vi "SoundInput-DAQ.vi"(7 "Name(\"\" to use uuid)":string="Acquisition") -> ()   [LabVIEW 2017, in "SoundInput-DAQ.lvlib"]
uses:
  SoundInput-DAQ.lvlib
  <vilib>/sound2/lvsound2.llb/Sound Data Format.ctl
  <vilib>/sound2/lvsound2.llb/Sampling Mode.ctl
  bc6f9ce3-7135-4df3-9fce-67397201bd09.vi
  15320dbe-bea9-49cb-a904-6d9e4fcf93d5.vi
  f3e3012a-dc83-45d7-82c5-490bef76f43f.vi
  e2413101-be31-4c43-921b-7e7496268bc5.vi
  07cbb487-6694-43fd-ac53-f2be3466fcff.vi
  fecb174d-6823-407c-a974-ffebb4610b14.vi
  0bf643a1-791c-4b4c-b91f-da80b9c7e2fb.vi
  041ba748-83ae-40d3-86c4-8e2f4b565384.vi
  <userlib>/_NEVSTOP/Communicable State Machine(CSM)/AdvanceAPI/CSM - Revert Arguments-Safe String.vi
  <userlib>/_NEVSTOP/Communicable State Machine(CSM)/_Shared/Trim Single-line Text.vi
  <userlib>/_NEVSTOP/Communicable State Machine(CSM)/AdvanceAPI/CSM - Make String Arguments Safe.vi
  <userlib>/_NEVSTOP/Communicable State Machine(CSM)/AdvanceAPI/CSM - Break Down Multiple States String.vi
  <userlib>/_NEVSTOP/Communicable State Machine(CSM)/AdvanceAPI/CSM - Compact Multiple States.vi
  f3e3012a-dc83-45d7-82c5-490bef76f43f.vi/99de0c97-112a-4c86-9094-c187659127e1.vi
  <userlib>/_NEVSTOP/Communicable State Machine(CSM)/Utility/Build Error Cluster.vi
  0bf643a1-791c-4b4c-b91f-da80b9c7e2fb.vi/99de0c97-112a-4c86-9094-c187659127e1.vi
  <userlib>/_NEVSTOP/Communicable State Machine(CSM)/AdvanceAPI/CSM - Keywords.vi
  <vilib>/Utility/Data Type/Get Type Information.vi
  <userlib>/_NEVSTOP/Communicable State Machine(CSM)/addons/API-String-Arugments-Support/_Support/Data To SingleElementsArray_csm.vi
  <userlib>/_NEVSTOP/Communicable State Machine(CSM)/addons/API-String-Arugments-Support/_Support/Data To API String Arguments.vi
  <userlib>/_NEVSTOP/Communicable State Machine(CSM)/addons/INI-Static-Variable-Support/_Support/Parse Used Session and Name.vi
  <userlib>/_NEVSTOP/Communicable State Machine(CSM)/addons/INI-Static-Variable-Support/_Support/INI-FGV(lvlibp).vi
  <userlib>/_NEVSTOP/Communicable State Machine(CSM)/addons/INI-Static-Variable-Support/_Support/Populate String with INI Variable.vi
  <userlib>/_NEVSTOP/Communicable State Machine(CSM)/addons/API-String-Arugments-Support/_Support/Convert API String Arguments to Data(variant).vi
  <userlib>/_NEVSTOP/Communicable State Machine(CSM)/addons/API-String-Arugments-Support/_Support/SingleElementsArray To Data_csm.vi
  <userlib>/_NEVSTOP/Communicable State Machine(CSM)/addons/API-String-Arugments-Support/_Support/Query Data as API String Arguments(variant).vi
  <vilib>/sound2/lvsound2.llb/Sound Input Read (DBL).vi
  <userlib>/_NEVSTOP/Communicable State Machine(CSM)/addons/MassData-Parameter/_support/FGV-MassData(lvlibp).vi
  <userlib>/_NEVSTOP/Communicable State Machine(CSM)/_Polymophic/Add State(s) to Queue By BOOL(Element).vi
  <userlib>/_NEVSTOP/Communicable State Machine(CSM)/_Polymophic/CSM - Filter Duplicated Lines.vi
  <userlib>/_NEVSTOP/Communicable State Machine(CSM)/_Polymophic/CSM - Replace Marks in Messages.vi
  <userlib>/_NEVSTOP/Communicable State Machine(CSM)/Communicable State Machine.lvlib
  <userlib>/_NEVSTOP/Communicable State Machine(CSM)/addons/Loop-Support/CSM Loop Support.lvlib
  <userlib>/_NEVSTOP/Communicable State Machine(CSM)/_Shared/CSM Shared.lvlib
panel:
  in  "Sound Format":T1={"sample rate (S/s)"=20000.0, "number of channels"=2, "bits per sample"=16}
  in  "Device ID":u32 format="%.0x"
  in  "SamplePeroid(ms)":i32=200
  out "Raw Data":waveform(dbl)[](graph)
  in  "Cancel Button":bool
  in  "OK Button":bool
  out "Error Occurred":errorcluster
  out "State History":string
  # "*(Windows) You must have DirectX 8.0 or later to use the Sound VIs. (Linux) You must have the Open Sound System (OSS) driver to use the Sound VIs."
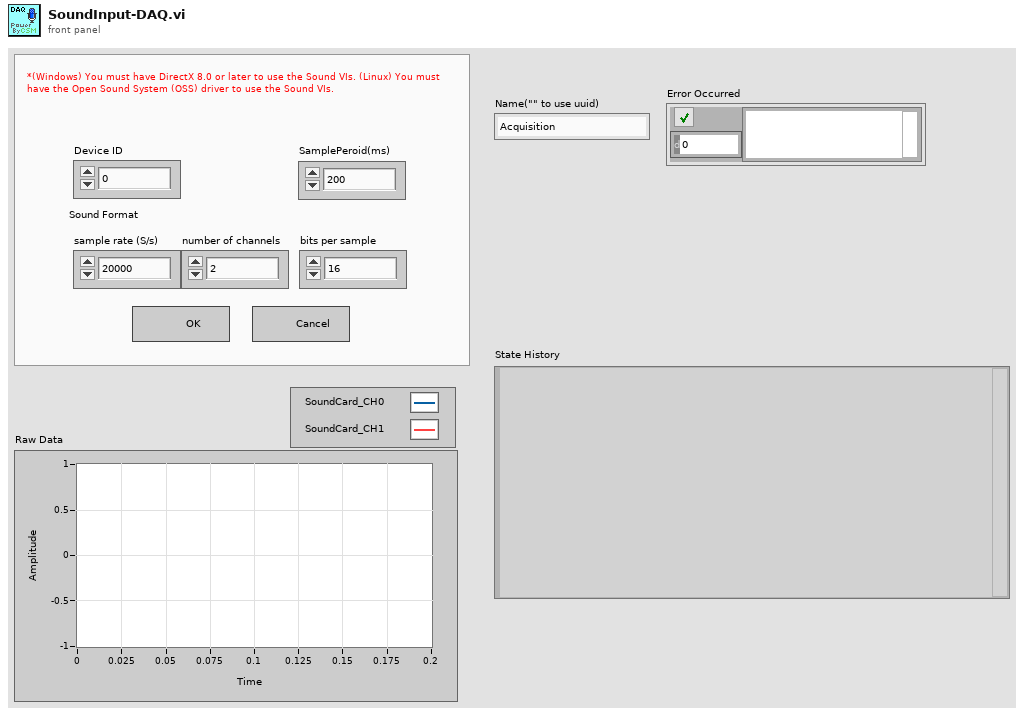
[diagram p1: front panel]
types:
  T1 = cluster{"sample rate (S/s)":dbl, "number of channels":i32, "bits per sample":i32}
  T2 = enum32{"Invalid", "Default", "Floating", "Floating/Auto-Hide", "Modal"}
  T3 = cluster{"Device ID":u32, "SamplePeroid(ms)":i32, "Sound Format":cluster{"sample rate (S/s)":dbl, "number of channels":i32, "bits per sample":i32}}
  T4 = enum32{"Invalid", "Standard", "Closed", "Hidden", "Minimized", "Maximized"}
  T5 = enum32{"invalid app kind", "Development System", "Run Time System", "Student Edition", "Embedded LabVIEW", "Evaluation", "Custom"}
  T6 = typedef "Communicable State Machine.lvlib/_CSM_Response Source Message.ctl" = cluster{"‘State":string, "’Arguments":string, "’Error":errorcluster}
  T7 = cluster{"Current VI Reference":refnum<vi>, "Close Panel on Exit?":bool}
  T8 = typedef "Sound Data Format.ctl" = cluster{"sample rate (S/s)":dbl, "number of channels":i32, "bits per sample":i32}
  T9 = cluster{"Core":cluster{"Current VI Reference":refnum<vi>, "Close Panel on Exit?":bool}, "Configuration":cluster{"Device ID":u32, "SamplePeroid(ms)":i32, "Sound Format":T8}, "State":enum16{"Idle", "Acquiring"}, "Number of Samples/ch":i32, "timestamp":timestamp}
  T10 = cluster{"Device ID":u32, "SamplePeroid(ms)":i32, "Sound Format":T8}
  T11 = typedef "Sampling Mode.ctl" = i32
  T12 = typedef "Sound Input Task ID.ctl" = u32
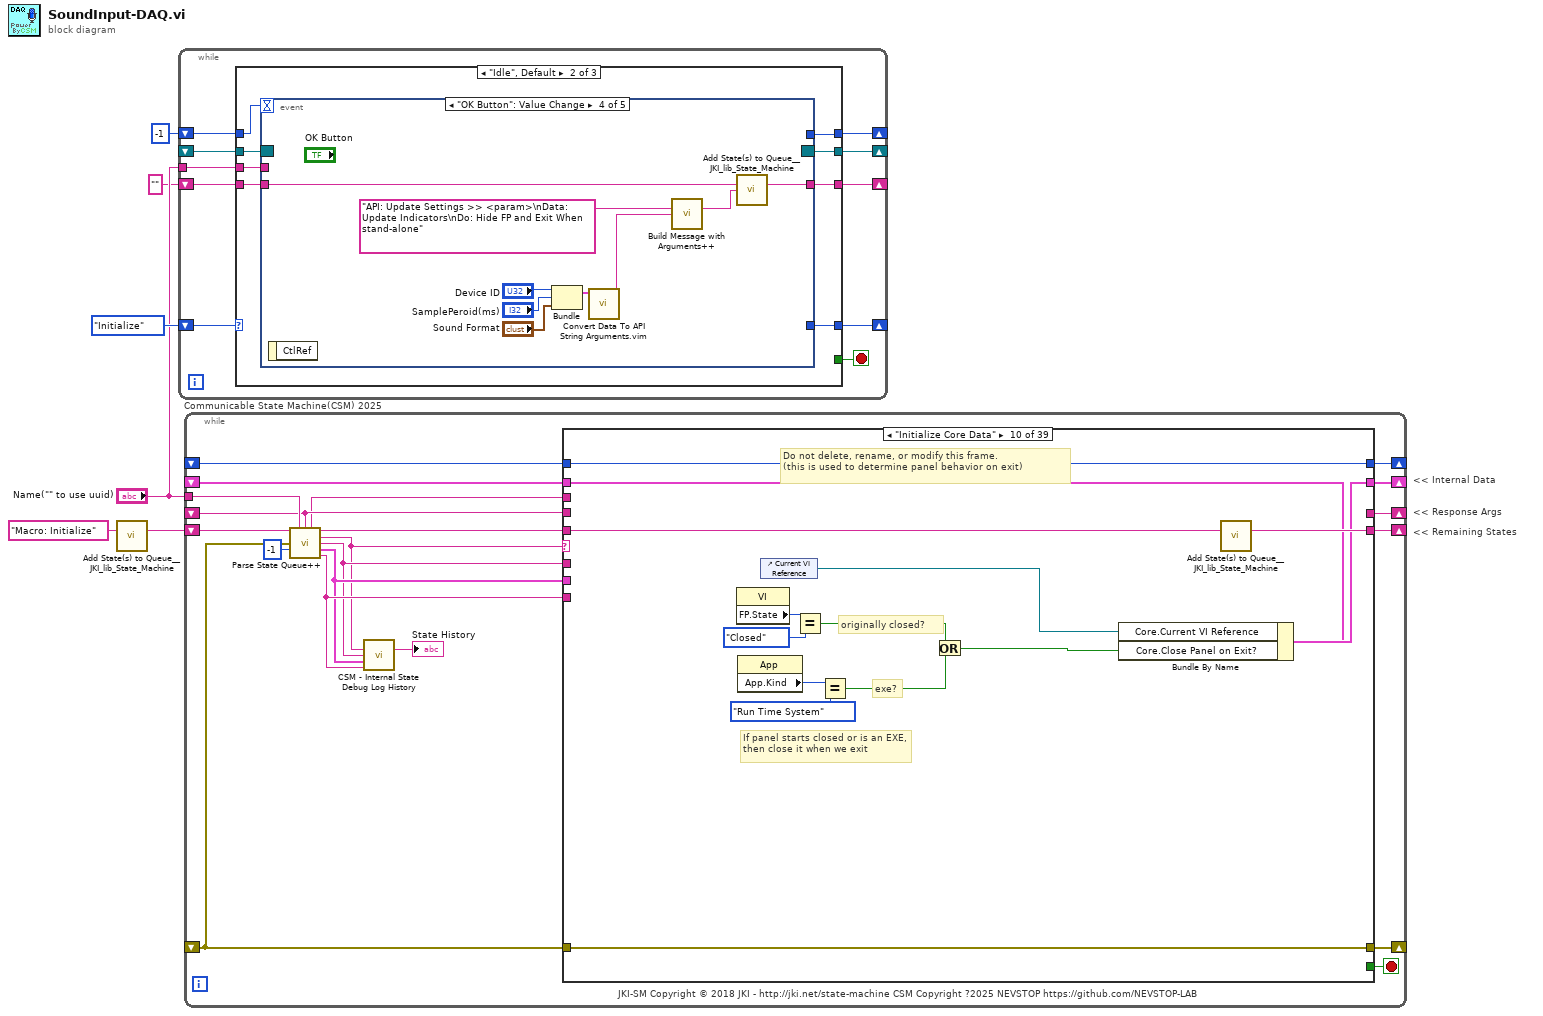
[diagram p0: block diagram]
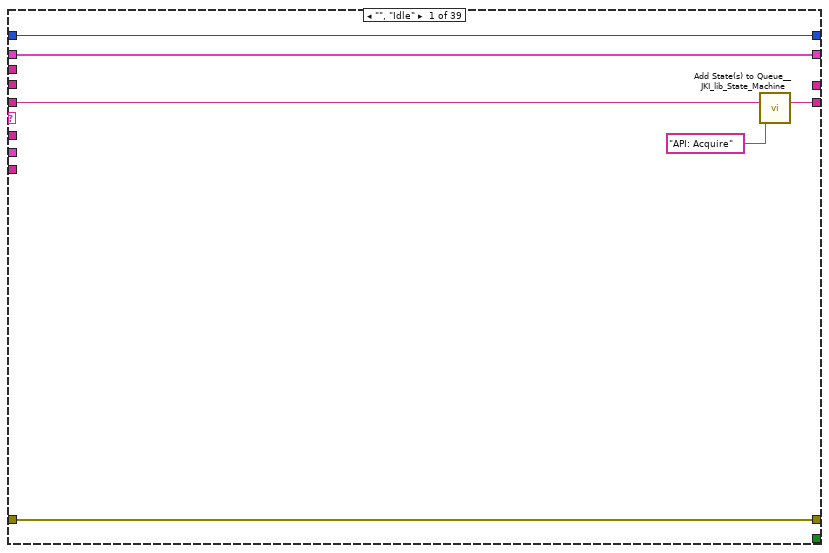
[diagram p2: hidden frame]
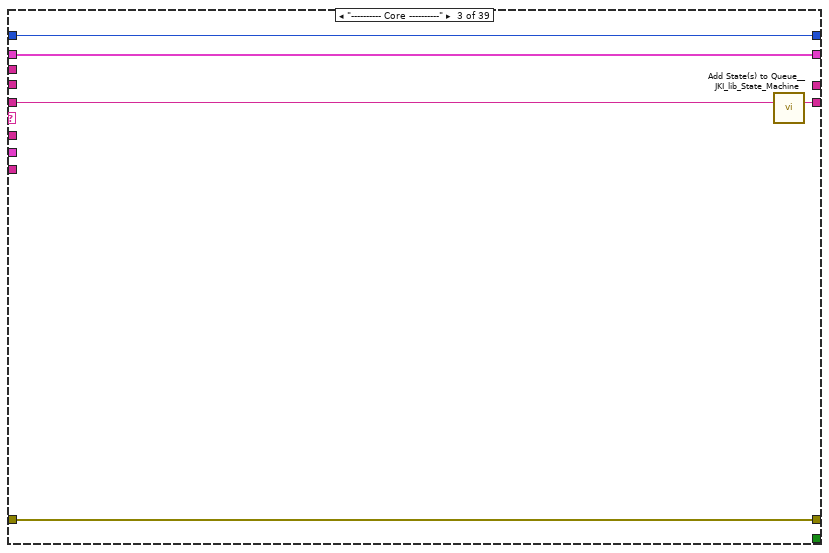
[diagram p4: hidden frame]
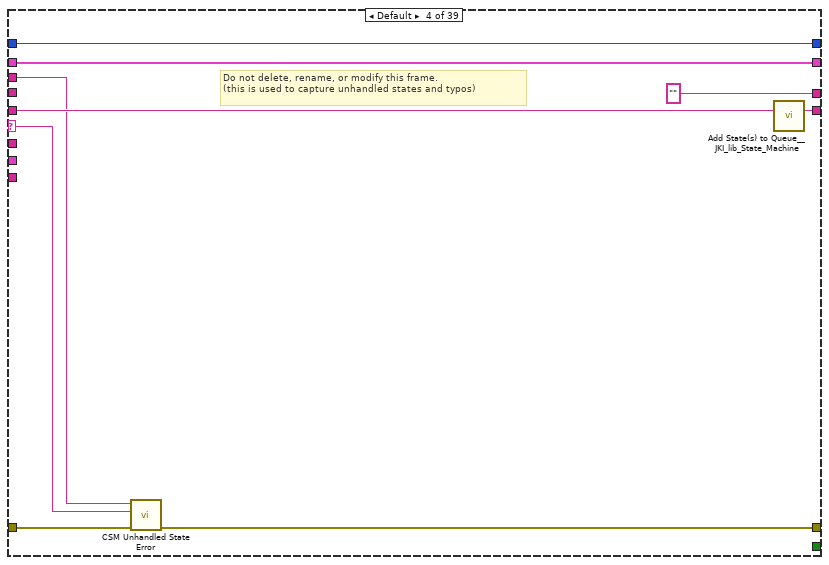
[diagram p5: hidden frame]
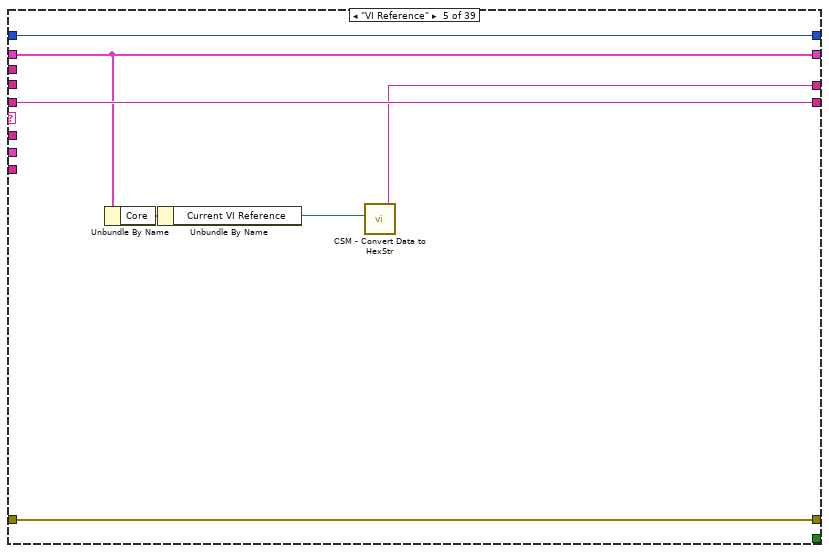
[diagram p6: hidden frame]
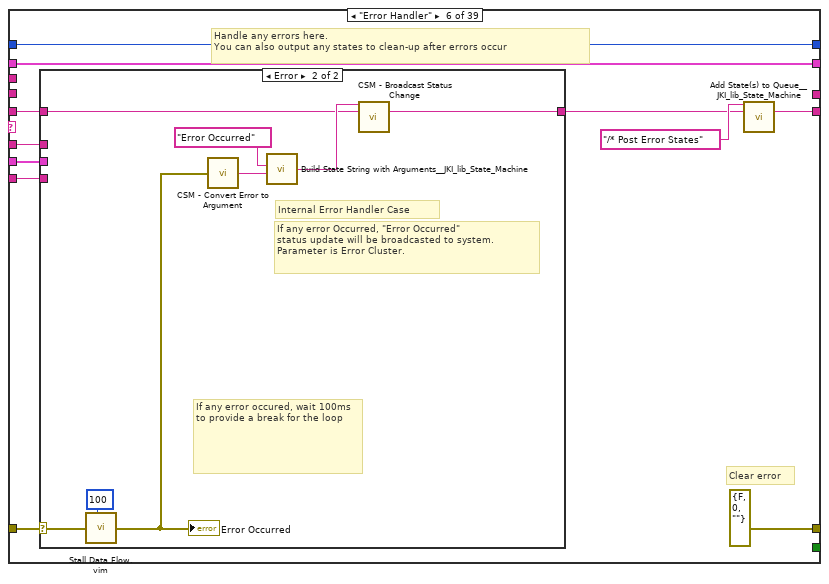
[diagram p7: hidden frame]
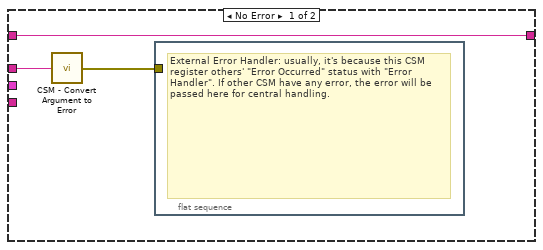
[diagram p8: hidden frame]
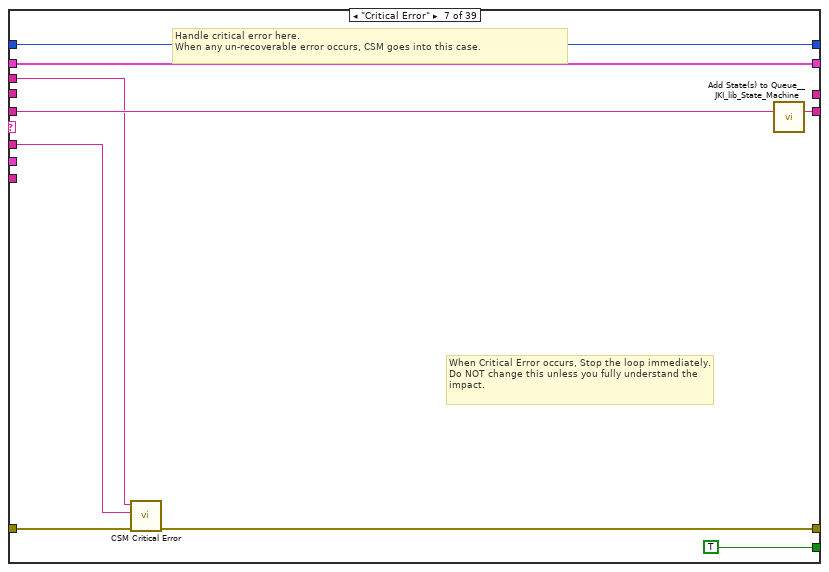
[diagram p9: hidden frame]
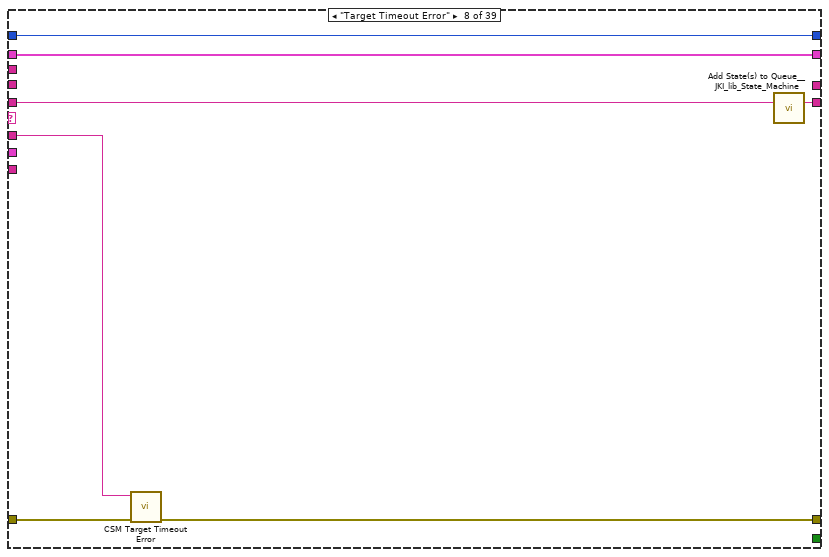
[diagram p10: hidden frame]
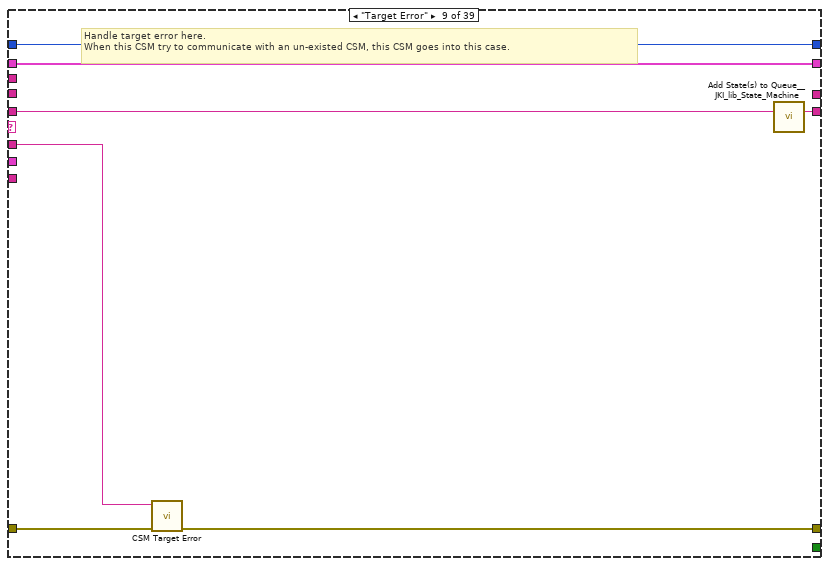
[diagram p11: hidden frame]
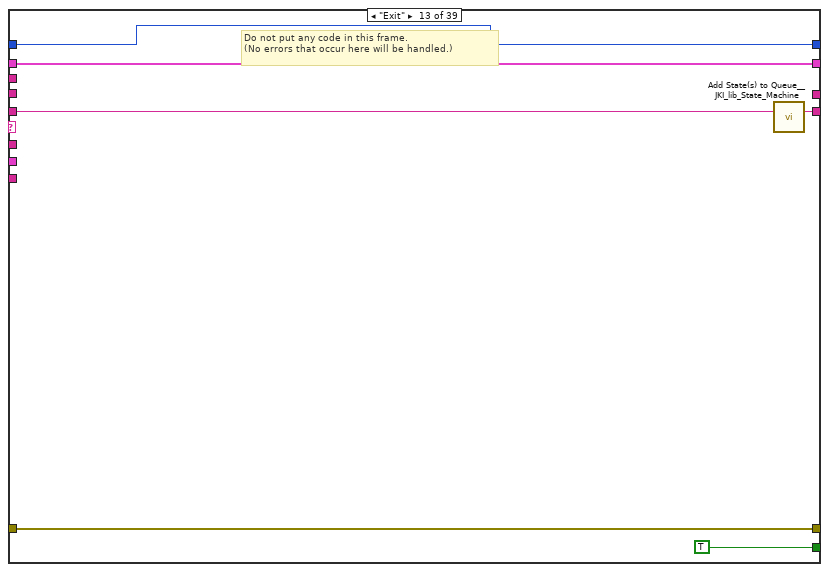
[diagram p14: hidden frame]
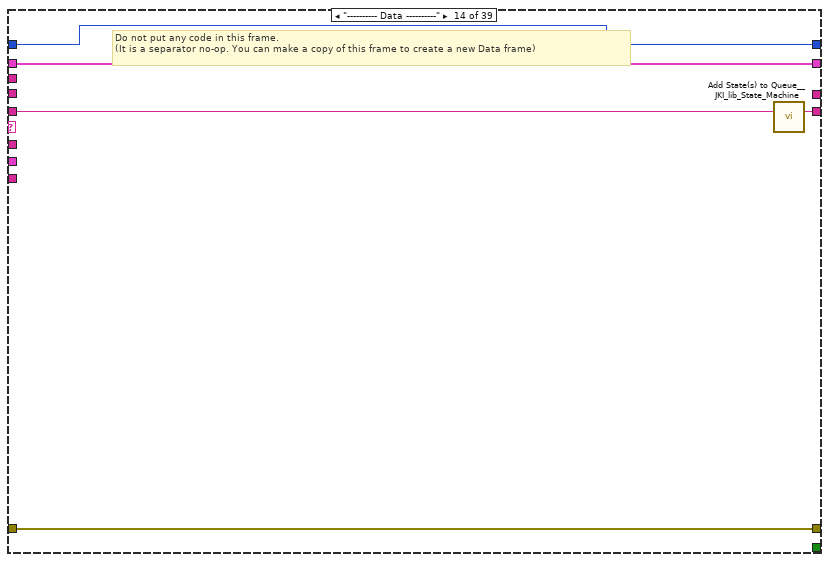
[diagram p15: hidden frame]
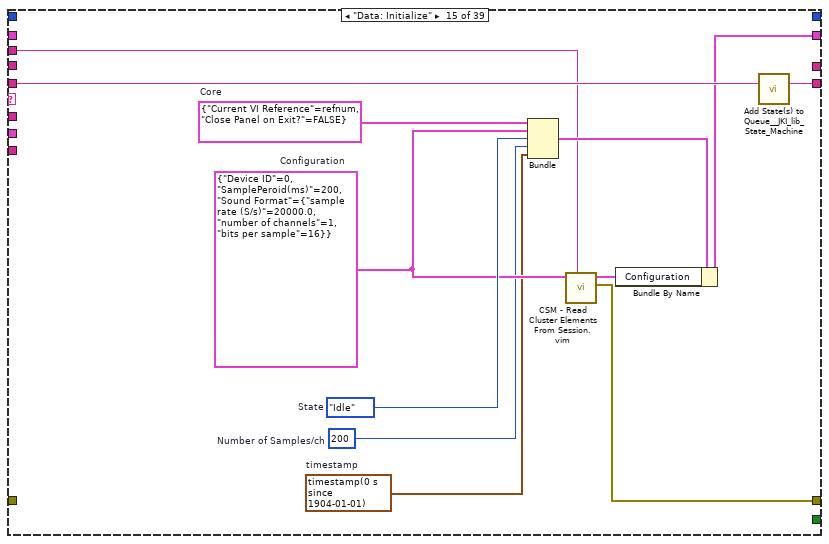
[diagram p16: hidden frame]
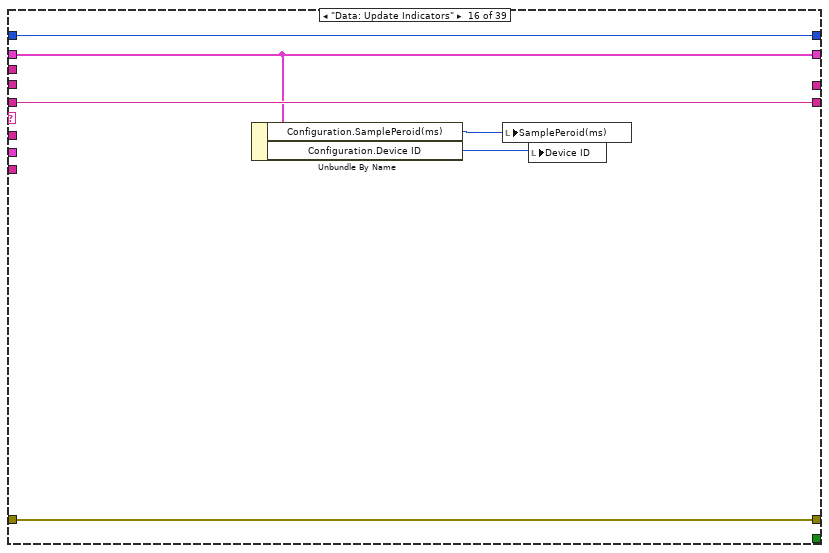
[diagram p17: hidden frame]
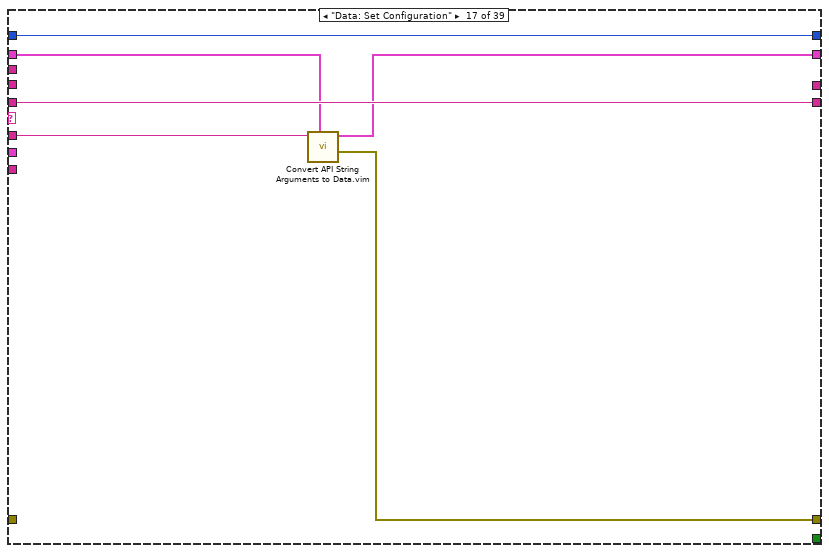
[diagram p18: hidden frame]
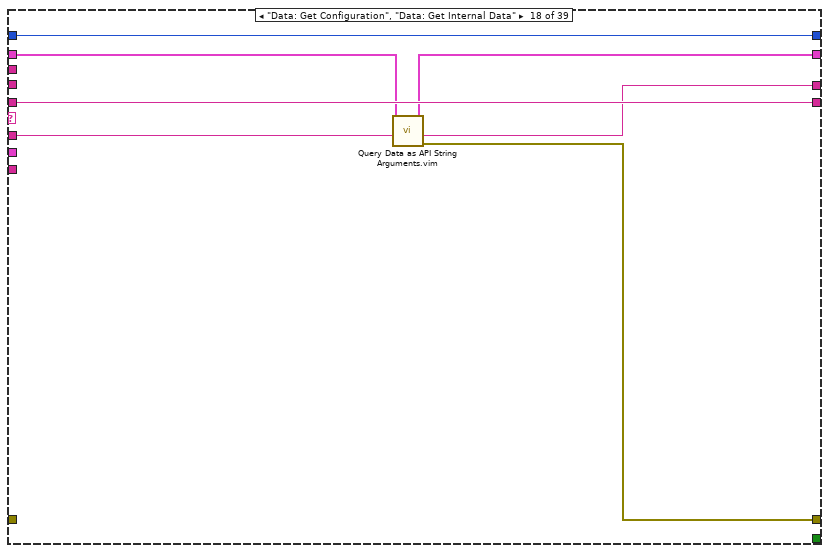
[diagram p19: hidden frame]
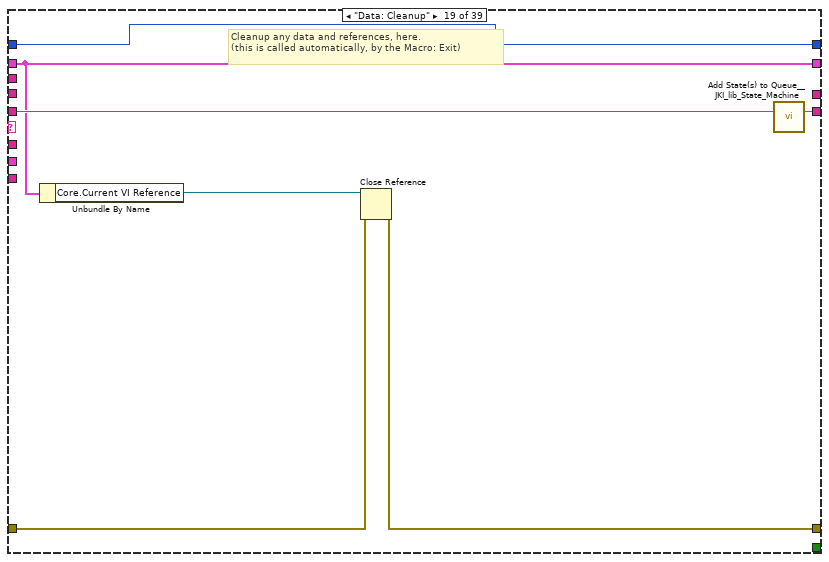
[diagram p20: hidden frame]
diagram:
  # "<< Internal Data"
  # "<< Response Args"
  # "<< Remaining States"
  n1 = call <vilib>:"Add State(s) to Queue__JKI_lib_State_Machine.vi"("State(s) in (\"\")"="Macro: Initialize") -> ("States Out"=w5:string)  [unwired: 14 in]
  n2 = while {
    shift-right: [w12] -> _
    shift-left: enum16{"Idle", "Initialize", "Exit"}."Initialize" -> [w16]
    tunnel: "Name(\"\" to use uuid)" -> [w15]
    shift-right: [w14] -> _
    shift-left: _ -> [w13]
    shift-right: [w9] -> _
    shift-left: "" -> [w10]
    shift-right: [w7] -> _
    shift-left: -1 -> [w8]
    stop <- w11 stop-if-true
    n3 = case shown="\"Idle\", Default" w16 {
      tunnel: w15 -> [w24 w27 _]
      tunnel: [w21 w32 _] -> w14
      tunnel: w13 -> [_ w31 w61]
      tunnel: [enum16{"Idle", "Initialize", "Exit"}."Idle" w30 _] -> w12
      tunnel: [_ _ TRUE] -> w11
      tunnel: w10 -> [w19 w29 w58]
      tunnel: [w19 w28 w58] -> w9
      tunnel: w8 -> [w18 w25 w57]
      tunnel: [w18 w26 w57] -> w7
      frame "Initialize" {
        n4 = call <userlib>:"CSM - Module Exit Event.vi"("Name (\"\" to Use UUID) In"=w24) -> ("error out"=w23:errorcluster, "CSM Exit Event"=w22:refnum<user-event>)  [unwired: 8 in, 1 out]
        n5 = register-events(error in=w23, w22) -> (reference out=w21:refnum<event-registration>)  [unwired: 1 in, 1 out]
        n6 = property class="VI"("FP.Behavior"=T2."Default" ("Front Panel Window:Behavior")) -> ()  [unwired: 2 in, 2 out]
      }
      frame "Idle", Default {
        n7 = event shown="[3] \"OK Button\": Value Change" {
          selector: w31 -> [_ _ _ _ _]
          dyn-events: [_ _ _ _ _] -> w32
          timeout: w25 -> [_ _ _ _ _]
          tunnel: [_ _ enum16{"Idle", "Initialize", "Exit"}."Exit" _ _] -> w30
          tunnel: w29 -> [w36 w40 w42 w52 w55]
          tunnel: [w37 w39 w42 w45 w54] -> w28
          tunnel: w27 -> [w34 _ _ _ _]
          tunnel: [-1 _ _ _ _] -> w26
          event Timeout {
            n8 = event-data() -> ()  [unwired: 1 in, 1 out]
            n9 = call-poly <userlib>:"CSM - Filter JKISM String Queue.vi"("States In"=w36) -> ("States Out"=w33:string)  [unwired: 14 in]
            n10 = call <userlib>:"CSM - Forward UI Operations to CSM.vi"("Name (\"\" to Use UUID)"=w34, "State(s) In (\"\")"=w33) -> ("States Out"=w37:string)  [unwired: 8 in, 1 out]
          }
          event Panel Close? {
            n11 = event-data() -> ()  [unwired: 1 in, 2 out]
            n12 = call <vilib>:"Add State(s) to Queue__JKI_lib_State_Machine.vi"("State(s) in (\"\")"=w40, "State(s) at Back (\"\")"="Do: Hide FP and Exit When stand-alone" ("State(s) at Back (\"\")")) -> ("States Out"=w39:string)  [unwired: 13 in]
            n13 = event-data("Discard?"=TRUE) -> ()  [unwired: 1 in, 1 out]
          }
          event User Event {
            n14 = event-data() -> ()  [unwired: 1 in, 1 out]
          }
          event "OK Button": Value Change {
            n15 = event-data() -> ()  [unwired: 1 in, 1 out]
            n16 = Bundle("Device ID"="Device ID", "SamplePeroid(ms)"="SamplePeroid(ms)", "Sound Format"="Sound Format") -> (w47:T3)  [unwired: 1 in]
            n17 = call "Convert Data To API String Arguments.vim"("Data"=w47) -> ("API String"=w50:string)  [unwired: 7 in, 1 out]
            n18 = call-poly <userlib>:"Build Message with Arguments++.vi"("States With Replace Token"="API: Update Settings >> <param>\nData: Update Indicators\nDo: Hide FP and Exit When stand-alone" ("State"), "<param>"=w50) -> ("States"=w44:string)  [unwired: 13 in]
            n19 = call <vilib>:"Add State(s) to Queue__JKI_lib_State_Machine.vi"("State(s) in (\"\")"=w52, "State(s) at Back (\"\")"=w44) -> ("States Out"=w45:string)  [unwired: 13 in]
          }
          event "Cancel Button": Value Change {
            n20 = event-data() -> ()  [unwired: 1 in, 1 out]
            n21 = call <vilib>:"Add State(s) to Queue__JKI_lib_State_Machine.vi"("State(s) in (\"\")"=w55, "State(s) at Back (\"\")"="Do: Hide FP and Exit When stand-alone" ("State(s) at Back (\"\")")) -> ("States Out"=w54:string)  [unwired: 13 in]
          }
        }
      }
      frame "Exit" {
        n22 = Unregister For Events(event registration refnum=w61) -> (error out=w60:errorcluster)  [unwired: 1 in]
        n23 = call <vilib>:"Clear Errors.vi"("error in (no error)"=w60) -> ()  [unwired: 5 in, 2 out]
        n24 = property class="VI"("FP.Behavior"=T2."Default" ("Front Panel Window:Behavior")) -> ()  [unwired: 2 in, 2 out]
      }
    }
  }
  n25 = while "Communicable State Machine(CSM) 2025" {
    shift-right: [w76] -> _
    shift-left: _ -> [w66]
    shift-right: [w79] -> _
    shift-left: _ -> [w75]
    shift-right: [w78] -> _
    shift-left: w5 -> [w80]
    tunnel: "Name(\"\" to use uuid)" -> [w73]
    shift-right: [w74] -> _
    shift-left: _ -> [w68]
    shift-right: [w63] -> _
    shift-left: _ -> [w62]
    stop <- w77 stop-if-true
    # "JKI-SM Copyright © 2018 JKI - http://jki.net/state-machine CSM Copyright ?2025 NEVSTOP https://github.com/NEVSTOP-LAB"
    n26 = call <userlib>:"Parse State Queue++.vi"("State Queue"=w80, "Name (\"\" to Use UUID)"=w73, "Response Arguments"=w68, "Previous Error"=w75, "Dequeue (1 ms)"=-1 ("Dequeue Timeout(1ms)")) -> ("Name Used"=w67:string, "Remaining States"=w81:string, "Current State"=w69:string, "Arguments"=w70:string, "Additional Information"=w71:T6, "Source CSM"=w72:string)  [unwired: 5 in]
    n27 = call <userlib>:"CSM - Internal State Debug Log History.vi"("State"=w69, "Arguments (\"\")"=w70, ">> Response Source Message >>"=w71, "Source (\"\")"=w72) -> ("Debug Log"=→"State History":string)  [unwired: 11 in]
    n28 = case shown="\"Initialize Core Data\"" w69 {
      selector: w69 -> [_ _ _ w98 _ _ _ _ _ _ _ _ _ _ _ _ _ _ _ _ _ _ _ _ _ _ _ _ _ _ _ _ _ _ w372 _ _ _ _]
      tunnel: w81 -> [w84 w90 w96 w104 w111 w117 w142 w149 w156 w171 w174 w178 w185 w190 w202 w207 w214 w221 w228 w233 w239 w245 w248 w253 w267 w281 w293 w307 w310 w315 w326 w359 w364 w367 w375 w384 w389 w397 w468]
      tunnel: w70 -> [_ _ _ _ _ w116 w136 w145 w152 _ _ _ _ _ _ _ w212 w218 _ _ _ _ _ _ _ w277 _ _ _ _ _ _ _ _ w371 _ _ w394 _]
      tunnel: w66 -> [w86 w89 w93 w102 w110 w122 w140 w147 w154 w164 w173 w177 w183 w187 _ w205 w213 w220 w223 w230 w236 w242 w247 w256 w263 w279 w292 w306 w308 w314 w328 w358 w363 w366 w373 w385 w388 w396 w473]
      tunnel: [w87 w91 w94 w97 w112 errorcluster {"status"=FALSE, "code"=0, "source"=""} ("error out") w135 w144 w151 w168 w175 w179 w182 w188 w193 w208 w210 w216 w224 w231 w237 w243 w249 w254 w265 w273 w294 w303 _ w316 w330 _ w360 w368 w376 w386 w390 w393 w474] -> w79
      tunnel: w75 -> [w87 w91 w94 w105 w112 w120 w143 w150 w157 w168 w175 w179 w182 w188 _ w208 _ _ w225 w231 w237 w243 w249 w254 w265 _ w294 _ _ w316 w331 _ _ w368 w376 w386 w390 w395 w474]
      tunnel: [w85 w90 w95 w103 w111 w118 w141 w148 w155 w170 w174 w178 w184 w189 w201 w207 w214 w221 w227 w232 w238 w244 w248 w252 w266 w281 w293 w307 w310 w315 w327 w359 w364 w367 w374 w383 w389 w397 w469] -> w78
      tunnel: [_ _ _ _ _ _ TRUE _ _ _ _ _ TRUE _ _ _ _ _ _ _ _ _ _ _ _ _ _ _ _ _ _ _ _ _ _ _ _ _ _] -> w77
      tunnel: [w86 w89 w93 w102 w110 w122 w140 w147 w154 w169 w173 w177 w183 w187 w195 w205 w211 w219 w223 w230 w236 w242 w247 w255 w263 w280 w292 w296 w308 w312 w329 w357 w363 w366 w369 w385 w388 w396 w473] -> w76
      tunnel: w72 -> [_ _ _ _ _ w115 _ _ _ _ _ _ _ _ _ _ _ _ _ _ _ _ _ _ _ _ _ _ _ _ _ _ _ _ _ _ _ _ _]
      tunnel: w71 -> [_ _ _ _ _ w114 _ _ _ _ _ _ _ _ _ _ _ _ _ _ _ _ _ _ _ _ _ _ _ _ _ _ _ _ _ _ _ _ _]
      tunnel: [_ _ _ "" w107 _ _ _ _ _ _ _ _ _ _ _ _ w217 _ _ _ _ _ _ _ _ _ _ _ _ w319 _ _ _ _ _ _ _ _] -> w74
      tunnel: w67 -> [_ _ _ w99 _ _ w137 _ _ _ _ _ _ _ w197 _ _ _ _ _ _ _ _ _ _ w272 _ _ _ _ _ _ _ _ _ _ _ _ _]
      tunnel: w68 -> [_ _ _ _ _ _ _ _ _ _ _ _ _ _ _ _ _ _ _ _ _ _ _ _ _ _ _ _ _ _ _ _ _ _ _ _ _ _ _]
      tunnel: [w82 w88 w92 w100 w106 w113 w138 w146 w153 w158 w172 w176 w180 w186 _ w204 w209 w215 w222 w229 w234 w240 w246 w250 w262 w270 w291 w302 w309 w313 w322 w355 _ w365 w370 w382 w387 w391 w472] -> w63
      tunnel: w62 -> [w82 w88 w92 w100 w106 w113 w138 w146 w153 w158 w172 w176 w180 w186 _ w204 w209 w215 w222 w229 w234 w240 w246 w250 w262 w270 w291 _ w309 w313 w323 w355 w362 w365 w370 w382 w387 w391 w472]
      frame "", "Idle" {
        n29 = call <vilib>:"Add State(s) to Queue__JKI_lib_State_Machine.vi"("State(s) in (\"\")"=w84, "State(s) at Back (\"\")"="API: Acquire" ("State(s) in Front (\"\")")) -> ("States Out"=w85:string)  [unwired: 13 in]
      }
      frame "CSM Documentation" {
        # "CSM Documentation"
        # "State Syntax:\nStateCategory: State >> Argument -@ CSMName\nStateCategory: State >> Argument -> CSMName\n\nLine Terminator: Line feed"
        # "Commenting:\nTo add a comment use \"//\" or \"#\" and all text to the right will be ignored\nCommenting Example:\nUI: Initialize // This initializes the UI\n// Another comment line"
        # "Example:\nUI: Help >> About -@Main\nUI: Help >> About ->Main\n\nWhere \"UI\" is the state category\nWhere \"Help\" is the state\nWhere \"About\" is the argument\nWhere \"Main\" is the Name of CSM,which actually run the \"UI: Help >> About\"\n\n    \"-@\" stands for sync state. Current CSM will wait until the state is finished. \n            - if \"Main\" named CSM does not exist, \"Target Error\" will occur.\n            - if \"Main\" named CSM is in another sync remote state, \"Target Busy Error\" will occur.\n            - if \"Main\" named CSM could not finish the state in time, \"Target Timeout Error\" will occur.\n            - if everything is right. \"Response\" will occur with Argument back from \"Main\" named CSM. \n\n    \"->\" stands for async state. Current CSM will post the state and continue to next state in next iteration.\n            - if \"Main\" named CSM does not exist, \"Target Error\" will occur.\n            - if everything is right. \"Async Message Posted\" will occur.\n            - After State is finished. Caller will receive a \"Async Response\" state from callee.\n\nWhen duplicated name is used for multiple CSM module or some framework problem happens, \"Critical Error\" will occur."
      }
      frame "---------- Core ----------" {
        n30 = call <vilib>:"Add State(s) to Queue__JKI_lib_State_Machine.vi"("State(s) in (\"\")"=w96) -> ("States Out"=w95:string)  [unwired: 14 in]
      }
      frame Default {
        # "Do not delete, rename, or modify this frame.\n(this is used to capture unhandled states and typos)"
        n31 = call <userlib>:"CSM Unhandled State Error.vi"("error in (no error)"=w105, "Undefined State"=w98, "CSM Name"=w99) -> ("error out"=w97:errorcluster)  [unwired: 8 in]
        n32 = call <vilib>:"Add State(s) to Queue__JKI_lib_State_Machine.vi"("State(s) in (\"\")"=w104) -> ("States Out"=w103:string)  [unwired: 14 in]
      }
      frame "VI Reference" {
        n33 = Unbundle By Name(w110) -> ("Core"=w109:T7)
        n34 = Unbundle By Name(w109) -> ("Current VI Reference"=w108:refnum<vi>)
        n35 = call <userlib>:"CSM - Convert Data to HexStr.vi"("Variant"=w108) -> ("HEX String (0-9,A-F)"=w107:string)  [unwired: 8 in]
      }
      frame "Error Handler" {
        # "Handle any errors here.\nYou can also output any states to clean-up after errors occur"
        # "Clear error"
        n36 = case shown="Error" w120 {
          selector: w120 -> [_ w129]
          tunnel: [w126 w131] -> w119
          tunnel: w117 -> [w126 w130]
          tunnel: w116 -> [w125 _]
          tunnel: w115 -> [_ _]
          tunnel: w114 -> [_ _]
          frame No Error {
            n37 = call <userlib>:"CSM - Convert Argument to Error.vi"("Argument"=w125) -> ("Error"=w124:errorcluster)  [unwired: 4 in]
            n38 = flat-sequence {
              tunnel: w124 -> [_]
              frame #0 {
                # "External Error Handler: usually, it's because this CSM register others' \"Error Occurred\" status with \"Error Handler\". If other CSM have any error, the error will be passed here for central handling."
              }
            }
          }
          frame Error {
            # "If any error occured, wait 100ms to provide a break for the loop"
            # "Internal Error Handler Case"
            # "If any error Occurred, \"Error Occurred\" \nstatus update will be broadcasted to system.\nParameter is Error Cluster."
            n39 = call "Stall Data Flow.vim"("value in"=w129, "milliseconds to wait"=u32 100) -> ("value out"=w128:errorcluster)  [unwired: 1 out]
            "Error Occurred" <- w128
            n40 = call <userlib>:"CSM - Convert Error to Argument.vi"("Error"=w128) -> ("Argument"=w133:string)  [unwired: 4 in]
            n41 = call <vilib>:"Build State String with Arguments__JKI_lib_State_Machine.vi"("Arguments (\"\")"=w133, "State"="Error Occurred" ("Status with Arguments")) -> ("State with Arguments"=w132:string)  [unwired: 4 in]
            n42 = call <userlib>:"CSM - Broadcast Status Change.vi"("Status With Arguments"=w132, "State Queue"=w130) -> ("Remaining States"=w131:string)  [unwired: 13 in]
          }
        }
        n43 = call <vilib>:"Add State(s) to Queue__JKI_lib_State_Machine.vi"("State(s) in Front (\"\")"="/* Post Error States", "State(s) in (\"\")"=w119) -> ("States Out"=w118:string)  [unwired: 13 in]
      }
      frame "Critical Error" {
        # "Handle critical error here.\nWhen any un-recoverable error occurs, CSM goes into this case."
        # "When Critical Error occurs, Stop the loop immediately. Do NOT change this unless you fully understand the impact."
        n44 = call <userlib>:"CSM Critical Error.vi"("error in (no error)"=w143, "Arugments (As Reason)"=w136, "CSM Name"=w137) -> ("error out"=w135:errorcluster)  [unwired: 8 in]
        n45 = call <vilib>:"Add State(s) to Queue__JKI_lib_State_Machine.vi"("State(s) in (\"\")"=w142) -> ("States Out"=w141:string)  [unwired: 14 in]
      }
      frame "Target Timeout Error" {
        n46 = call <userlib>:"CSM Target Timeout Error.vi"("error in (no error)"=w150, "Arguments (As CSM Name)"=w145) -> ("error out"=w144:errorcluster)  [unwired: 9 in]
        n47 = call <vilib>:"Add State(s) to Queue__JKI_lib_State_Machine.vi"("State(s) in (\"\")"=w149) -> ("States Out"=w148:string)  [unwired: 14 in]
      }
      frame "Target Error" {
        # "Handle target error here.\nWhen this CSM try to communicate with an un-existed CSM, this CSM goes into this case."
        n48 = call <userlib>:"CSM Target Error.vi"("error in (no error)"=w157, "Arguments (As CSM Name)"=w152) -> ("error out"=w151:errorcluster)  [unwired: 9 in]
        n49 = call <vilib>:"Add State(s) to Queue__JKI_lib_State_Machine.vi"("State(s) in (\"\")"=w156) -> ("States Out"=w155:string)  [unwired: 14 in]
      }
      frame "Initialize Core Data" {
        # "Do not delete, rename, or modify this frame.\n(this is used to determine panel behavior on exit)"
        # "originally closed?"
        # "exe?"
        # "If panel starts closed or is an EXE, then close it when we exit"
        n50 = property class="VI"() -> ("FP.State"=w161:T4)  [unwired: 2 in, 2 out]
        n51 = property class="App"() -> ("App.Kind"=w167:T5)  [unwired: 2 in, 2 out]
        n52 = control-ref of="Current VI Reference"() -> (w162:refnum<vi>)
        n53 = Equal?(x=w161, y=T4."Closed" ("Front Panel Window:State")) -> (x = y?=w159:bool)
        n54 = Equal?(x=w167, y=T5."Run Time System" ("Application:Kind")) -> (x = y?=w165:bool)
        n55 = Or(x=w159, y=w165) -> (x .or. y?=w163:bool)
        n56 = Bundle By Name(cluster=w164, "Core.Current VI Reference"=w162, "Core.Close Panel on Exit?"=w163) -> (w169:T9)
        n57 = call <vilib>:"Add State(s) to Queue__JKI_lib_State_Machine.vi"("State(s) in (\"\")"=w171) -> ("States Out"=w170:string)  [unwired: 14 in]
      }
      frame "Async Response", "Response" {
      }
      frame "Async Message Posted" {
      }
      frame "Exit" {
        # "Do not put any code in this frame.\n(No errors that occur here will be handled.)"
        n58 = call <vilib>:"Add State(s) to Queue__JKI_lib_State_Machine.vi"("State(s) in (\"\")"=w185) -> ("States Out"=w184:string)  [unwired: 14 in]
      }
      frame "---------- Data ----------" {
        # "Do not put any code in this frame.\n(It is a separator no-op. You can make a copy of this frame to create a new Data frame)"
        n59 = call <vilib>:"Add State(s) to Queue__JKI_lib_State_Machine.vi"("State(s) in (\"\")"=w190) -> ("States Out"=w189:string)  [unwired: 14 in]
      }
      frame "Data: Initialize" {
        w191 = timestamp(0 s since 1904-01-01)  # timestamp
        w192 = 200  # Number of Samples/ch
        w198 = enum16{"Idle", "Acquiring"}."Idle"  # State
        w196 = T10 {"Device ID"=0, "SamplePeroid(ms)"=200, "Sound Format"={"sample rate (S/s)"=20000.0, "number of channels"=1, "bits per sample"=16}}  # Configuration
        w199 = T7 {"Current VI Reference"=refnum, "Close Panel on Exit?"=FALSE}  # Core
        n60 = Bundle("Core"=w199, "Configuration"=w196, "State"=w198, "Number of Samples/ch"=w192, "timestamp"=w191) -> (w200:T9)  [unwired: 1 in]
        n61 = call "CSM - Read Cluster Elements From Session.vim"("Section Name (\"\" as Default)"=w197, "Cluster"=w196) -> ("error out"=w193:errorcluster, "Cluster out"=w194:T10)  [unwired: 6 in]
        n62 = Bundle By Name(cluster=w200, "Configuration"=w194) -> (w195:T9)
        n63 = call <vilib>:"Add State(s) to Queue__JKI_lib_State_Machine.vi"("State(s) in (\"\")"=w202) -> ("States Out"=w201:string)  [unwired: 14 in]
      }
      frame "Data: Update Indicators" {
        n64 = Unbundle By Name(w205) -> ("Configuration.SamplePeroid(ms)"=w206:i32, "Configuration.Device ID"=w203:u32)
        n65 = local write "SamplePeroid(ms)"(w206) -> ()
        n66 = local write "Device ID"(w203) -> ()
      }
      frame "Data: Set Configuration" {
        n67 = call "Convert API String Arguments to Data.vim"("Reference Type"=w213, "API String"=w212) -> ("error out"=w210:errorcluster, "Data"=w211:T9)  [unwired: 6 in]
      }
      frame "Data: Get Configuration", "Data: Get Internal Data" {
        n68 = call "Query Data as API String Arguments.vim"("Name"=w218, "Cluster Data"=w220) -> ("error"=w216:errorcluster, "API String"=w217:string, "Cluster Data (dup)"=w219:T9)  [unwired: 7 in]
      }
      frame "Data: Cleanup" {
        # "Cleanup any data and references, here.\n(this is called automatically, by the Macro: Exit)"
        n69 = Unbundle By Name(w223) -> ("Core.Current VI Reference"=w226:refnum<vi>)
        n70 = Close Reference(reference=w226, error in (no error)=w225) -> (error out=w224:errorcluster)
        n71 = call <vilib>:"Add State(s) to Queue__JKI_lib_State_Machine.vi"("State(s) in (\"\")"=w228) -> ("States Out"=w227:string)  [unwired: 14 in]
      }
      frame "---------- Macro ----------" {
        # "Do not put any code in this frame.\n(It is a separator no-op. You can make a copy of this frame to create a new Macro frame)"
        n72 = call <vilib>:"Add State(s) to Queue__JKI_lib_State_Machine.vi"("State(s) in (\"\")"=w233) -> ("States Out"=w232:string)  [unwired: 14 in]
      }
      frame "Macro: Initialize" {
        n73 = call <vilib>:"Add State(s) to Queue__JKI_lib_State_Machine.vi"("State(s) in Front (\"\")"="Data: Initialize\nInitialize Core Data\nData: Update Indicators", "State(s) in (\"\")"=w239) -> ("States Out"=w238:string)  [unwired: 13 in]
      }
      frame "Macro: Exit" {
        w241 = "//Try to close device if needed\nDAQ: Close\n\nData: Cleanup\nExit"  # //Try to close device if needed DAQ: Close  Data: Cleanup Exit
        n74 = call <vilib>:"Add State(s) to Queue__JKI_lib_State_Machine.vi"("State(s) in Front (\"\")"=w241, "State(s) in (\"\")"=w245) -> ("States Out"=w244:string)  [unwired: 13 in]
      }
      frame "---------- API ----------" {
      }
      frame "API: Start" {
        # "#CSM-NOTE\nhttps://github.com/NEVSTOP-LAB/CSM-Continuous-Meausrement-and-Logging/issues/21\n\nUse CSM-Loop Support to define a loop in CSM, which is recommanded."
        n75 = Unbundle By Name(w256) -> ("State"=w257:enum16{"Idle", "Acquiring"})
        n76 = case shown="\"Acquiring\"" w257 {
          selector: w257 -> [w259 _]
          tunnel: [w259 enum16{"Idle", "Acquiring"}."Acquiring" ("Acquisition State")] -> w258
          tunnel: [_ "DAQ: Initialize \nDAQ: Configure\nDAQ: Start\nDAQ: Acquisite\nContinuous Check >> DAQ: Acquisite -><loop> \nDAQ: Stop\nDAQ: Close " ("State(s) in Front (\"\")")] -> w251
          frame "Acquiring" {
            # "The system is already acquiring. Ignore the \"Start\" message."
          }
          frame "Idle" {
            # "If the system is idle, start the acquisition."
          }
        }
        n77 = call <userlib>:"CSMLS - Define Loop State(s).vi"("Loop States"=w251, "States Queue"=w253) -> ("Remaining States"=w252:string)  [unwired: 13 in]
        n78 = Bundle By Name(cluster=w256, "State"=w258) -> (w255:T9)
      }
      frame "API: Stop" {
        # "Copy/Rename this case for your own API"
        n79 = Unbundle By Name(w263) -> ("State"=w268:enum16{"Idle", "Acquiring"})
        n80 = case shown="\"Acquiring\"" w268 {
          tunnel: ["Break Continuous" ("State(s) in Front (\"\")") _] -> w264
          frame "Acquiring" {
            # "If the system is acquiring, stop the acquisition."
          }
          frame "Idle" {
            # "The system is already idle. Ignore the \"Stop\" message."
          }
        }
        n81 = call <vilib>:"Add State(s) to Queue__JKI_lib_State_Machine.vi"("State(s) in Front (\"\")"=w264, "State(s) in (\"\")"=w267) -> ("States Out"=w266:string)  [unwired: 13 in]
      }
      frame "API: Update Settings" {
        # "#CSM-NOTE\nSync with ini-variable, to make sure the configuration could be stored in CSM INI-Variable configuration file."
        # "#CSM-NOTE\nUse this method to identify the argument type."
        n82 = Unbundle By Name(w279) -> ("Configuration"=w278:T10)
        n83 = call <userlib>:"CSM - Argument Type.vi"("Arguments"=w277) -> ("Argument Type"=w274:string, "Arguments (Dup)"=w275:string)  [unwired: 3 in]
        n84 = case shown="\"HexStr\"" w274 {
          tunnel: w278 -> [w284 w290]
          tunnel: [w283 w289] -> w271
          tunnel: [w282 w288] -> w276
          tunnel: w275 -> [w286 w287]
          frame "HexStr" {
            n85 = call <userlib>:"CSM - Convert HexStr to Data.vi"("HEX String"=w286) -> ("Variant"=w285:variant)  [unwired: 7 in, 1 out]
            n86 = Variant To Data(type=w284, Variant=w285) -> (data=w283:T10, error out=w282:errorcluster)  [unwired: 1 in]
          }
          frame Default {
            n87 = call "Convert API String Arguments to Data.vim"("Reference Type"=w290, "API String"=w287) -> ("error out"=w288:errorcluster, "Data"=w289:T10)  [unwired: 6 in]
          }
        }
        n88 = call "CSM - Write Configuration Variable.vim"("Section Name (\"\" as Default)"=w272, "error in (no error)"=w276, "Configuration"=w271) -> ("error out"=w273:errorcluster)  [unwired: 5 in, 1 out]
        n89 = Bundle By Name(cluster=w279, "Configuration"=w271) -> (w280:T9)
      }
      frame "---------- DAQ ----------" {
      }
      frame "DAQ: Initialize" {
        w305 = T11 1 items=["Finite Samples", "Continuous Samples"] ("sample mode")
        n90 = Unbundle By Name(w306) -> ("Configuration.Device ID"=w304:u32, "Configuration.SamplePeroid(ms)"=w301:i32, "Configuration.Sound Format"=w299:T8)
        n91 = Unbundle By Name(w299) -> ("sample rate (S/s)"=w298:dbl)
        n92 = Divide(x=1000, y=w301) -> (x/y=w297:dbl)
        n93 = Divide(x=w298, y=w297) -> (x/y=w295:dbl)
        n94 = Bundle By Name(cluster=w306, "Number of Samples/ch"=w295) -> (w296:T9)
        n95 = call <vilib>:"Sound Input Configure.vi"("number of samples/ch"=w295, "sample mode"=w305, "sound format"=w299, "device ID"=w304) -> ("error out"=w303:errorcluster, "task ID"=w302:T12)  [unwired: 6 in]
      }
      frame "DAQ: Configure" {
      }
      frame "DAQ: Start" {
        n96 = Get Date/Time In Seconds() -> (seconds since 1Jan1904=w311:timestamp)
        n97 = Bundle By Name(cluster=w314, "timestamp"=w311) -> (w312:T9)
      }
      frame "DAQ: Acquisite" {
        n98 = Unbundle By Name(w328) -> ("Number of Samples/ch"=w321:i32, "State"=w332:enum16{"Idle", "Acquiring"}, "timestamp"=w320:timestamp)
        n99 = case shown="\"Acquiring\"" w332 {
          tunnel: [w335 w344] -> w330
          tunnel: w331 -> [w335 w343]
          tunnel: [w334 w346] -> w329
          tunnel: w328 -> [w334 w346]
          tunnel: [_ w345] -> w319
          tunnel: w323 -> [w333 w341]
          tunnel: [w333 w340] -> w322
          tunnel: w321 -> [_ w339]
          tunnel: w320 -> [_ w336]
          frame "Idle" {
            # "Ignore \"Acquire\" messages when the acquisition is idle."
          }
          frame "Acquiring" {
            # "Acquire more data while in the \"Acquiring\" state."
            n100 = call-poly <vilib>:"Sound Input Read.vi"("number of samples/ch"=w339, "error in (no error)"=w343, "task ID"=w341) -> ("error out"=w342:errorcluster, "data"=w338:waveform(dbl)[], "task ID out"=w340:T12)  [unwired: 6 in]
            n101 = for {
              tunnel: w338 -> [w353] mode=indexing
              tunnel: [w348] -> w337 mode=indexing
              tunnel: w336 -> [w347]
              i -> [w351]
              n102 = Format Into String(format string="SoundCard_CH%d" ("name"), w351) -> (resulting string=w349:string)  [unwired: 2 in, 1 out]
              n103 = Set Waveform Attribute(5:w349, 6:"NI_ChannelName" ("name"), 7:w353) -> (3:w352:waveform(dbl))  [unwired: 1 in, 2 out]
              n104 = Bundle By Name(cluster=w352, "t0"=w347) -> (w348:waveform(dbl))
            }
            "Raw Data" <- w337
            n105 = call "CSM - Convert MassData to Argument.vim"("error in (no error)"=w342, "Data"=w337) -> ("error out"=w344:errorcluster, "MassData Argument"=w345:string)  [unwired: 6 in]
          }
        }
        n106 = call <vilib>:"Build State String with Arguments__JKI_lib_State_Machine.vi"("Arguments (\"\")"=w319, "State"="Acquired Waveform" ("Status with Arguments")) -> ("State with Arguments"=w324:string)  [unwired: 4 in]
        n107 = Empty String/Path?(string/path=w319) -> (empty?=w318:bool)
        n108 = Not(x=w318) -> (.not. x?=w317:bool)
        n109 = call <userlib>:"CSM - Broadcast Status Change.vi"("Status With Arguments"=w324, "State Queue"=w326, "Broadcast? (T)"=w317) -> ("Remaining States"=w327:string)  [unwired: 12 in]
      }
      frame "DAQ: Stop" {
        n110 = Bundle By Name(cluster=w358, "State"=enum16{"Idle", "Acquiring"}."Idle" ("Acquisition State")) -> (w357:T9)
      }
      frame "DAQ: Close" {
        n111 = call <vilib>:"Sound Input Clear.vi"("task ID"=w362) -> ("error out"=w361:errorcluster)  [unwired: 10 in]
        n112 = call <vilib>:"Clear Errors.vi"("error in (no error)"=w361) -> ("error out"=w360:errorcluster)  [unwired: 5 in, 1 out]
      }
      frame "---------- Control Logic ----------" {
      }
      frame "Continuous Check" {
        n113 = in-place {
          n114 = in-place-cluster #1(w373) -> ("Configuration.SamplePeroid(ms)"=w378:i32, "timestamp"=w381:timestamp)
          n115 = Divide(x=w378, y=1000 ("x")) -> (x/y=w379:dbl)
          n116 = Add(x=w381, y=w379) -> (x+y=w380:timestamp)
          n117 = in-place-cluster #1("Configuration.SamplePeroid(ms)"=w378, "timestamp"=w380) -> (w369:T9)
        }
        n118 = call <userlib>:"CSMLS - Append Continuous State.vi"("Loop State(s) And Arguments"=w371, "Continous Arguments (\"\")"=w371, "Continous State"=w372, "States Queue"=w375) -> ("Remaining States"=w374:string)  [unwired: 7 in]
      }
      frame "Break Continuous" {
        n119 = call <userlib>:"CSMLS - Remove Loop Tag to Break.vi"("States Queue"=w384) -> ("Remaining States"=w383:string)  [unwired: 10 in]
      }
      frame "---------- DoSth ----------" {
      }
      frame "Do: Front Panel State" {
        n120 = Unbundle By Name(w396) -> ("Core.Current VI Reference"=w392:refnum<vi>)
        n121 = case shown="\"Hidden\", \"Hide\"" w394 {
          tunnel: w395 -> [w403 w418 w429 w442 w455]
          tunnel: [w405 w419 w431 w444 w457] -> w393
          tunnel: w392 -> [w404 w416 w430 w443 w456]
          frame "Open", "Standard", Default {
            w398 = T4."Standard" ("State")
            n122 = property class="VI"(reference=w404, error in=w403) -> (reference out=w401:refnum<vi>, error out=w402:errorcluster, "FP.State"=w400:T4)
            n123 = Not Equal?(x=w400, y=w398) -> (x != y?=w399:bool)
            n124 = case shown="True" w399 {
              tunnel: [w409 w411] -> w405
              tunnel: w402 -> [w408 w411]
              tunnel: w401 -> [w407 _]
              tunnel: w398 -> [w406 _]
              frame True {
                n125 = invoke class="VI" method="FP.Open"(reference=w407, error in=w408, "Activate"=TRUE, "State"=w406) -> (error out=w409:errorcluster)  [unwired: 1 in, 4 out]
              }
              frame False {
              }
            }
          }
          frame "Close", "Closed" {
            n126 = property class="VI"(reference=w416, error in=w418) -> (reference out=w415:refnum<vi>, error out=w417:errorcluster, "FP.State"=w413:T4)
            n127 = Not Equal?(x=w413, y=T4."Closed" ("Front Panel Window:State")) -> (x != y?=w412:bool)
            n128 = case shown="True" w412 {
              tunnel: [w420 w423] -> w419
              tunnel: w417 -> [w420 w422]
              tunnel: w415 -> [_ w421]
              frame False {
              }
              frame True {
                n129 = invoke class="VI" method="FP.Close"(reference=w421, error in=w422) -> (error out=w423:errorcluster)  [unwired: 1 in, 2 out]
              }
            }
          }
          frame "Hidden", "Hide" {
            w424 = T4."Hidden" ("State")
            n130 = property class="VI"(reference=w430, error in=w429) -> (reference out=w427:refnum<vi>, error out=w428:errorcluster, "FP.State"=w426:T4)
            n131 = Not Equal?(x=w426, y=w424) -> (x != y?=w425:bool)
            n132 = case shown="True" w425 {
              tunnel: [w435 w436] -> w431
              tunnel: w428 -> [w434 w436]
              tunnel: w427 -> [w433 _]
              tunnel: w424 -> [w432 _]
              frame True {
                n133 = invoke class="VI" method="FP.Open"(reference=w433, error in=w434, "State"=w432) -> (error out=w435:errorcluster)  [unwired: 2 in, 4 out]
              }
              frame False {
              }
            }
          }
          frame "Minimize", "Minimized" {
            w437 = T4."Minimized" ("State")
            n134 = property class="VI"(reference=w443, error in=w442) -> (reference out=w440:refnum<vi>, error out=w441:errorcluster, "FP.State"=w439:T4)
            n135 = Not Equal?(x=w439, y=w437) -> (x != y?=w438:bool)
            n136 = case shown="True" w438 {
              tunnel: [w448 w449] -> w444
              tunnel: w441 -> [w447 w449]
              tunnel: w440 -> [w446 _]
              tunnel: w437 -> [w445 _]
              frame True {
                n137 = invoke class="VI" method="FP.Open"(reference=w446, error in=w447, "State"=w445) -> (error out=w448:errorcluster)  [unwired: 2 in, 4 out]
              }
              frame False {
              }
            }
          }
          frame "Maximize", "Maximized" {
            w450 = T4."Maximized" ("State")
            n138 = property class="VI"(reference=w456, error in=w455) -> (reference out=w453:refnum<vi>, error out=w454:errorcluster, "FP.State"=w452:T4)
            n139 = Not Equal?(x=w452, y=w450) -> (x != y?=w451:bool)
            n140 = case shown="True" w451 {
              tunnel: [w461 w462] -> w457
              tunnel: w454 -> [w460 w462]
              tunnel: w453 -> [w459 _]
              tunnel: w450 -> [w458 _]
              frame True {
                n141 = invoke class="VI" method="FP.Open"(reference=w459, error in=w460, "State"=w458) -> (error out=w461:errorcluster)  [unwired: 2 in, 4 out]
              }
              frame False {
              }
            }
          }
        }
      }
      frame "Do: Hide FP and Exit When stand-alone" {
        # "#CSM-NOTE\nNo parent"
        n142 = Call Chain() -> (call chain=w466:string[])
        n143 = Array Size(array=w466) -> (size(s)=w465:i32)
        n144 = Equal?(x=1, y=w465) -> (x = y?=w463:bool)
        n145 = call-poly <userlib>:"Add State(s) to Queue By BOOL++.vi"("TRUE (\"\")"="Macro: Exit" ("State(s) at Back (\"\")"), "Condition"=w463, "State Queue (\"\")"="Do: Front Panel State >> Hide" ("State(s) at Back (\"\")")) -> ("Remaining States"=w467:string)  [unwired: 8 in]
        n146 = call <vilib>:"Add State(s) to Queue__JKI_lib_State_Machine.vi"("State(s) in Front (\"\")"=w467, "State(s) in (\"\")"=w468) -> ("States Out"=w469:string)  [unwired: 13 in]
      }
    }
  }
